vi "Configure.vi"(4 "Results Folder":path, 5 "Verdict Display":refnum<vi>, 6 "Stopped Notification":refnum<notifier>, 7 "Step Table Display":refnum<vi>, 8 "error in":errorcluster, 9 "Step Index Display":refnum<vi>, 10 "Status Display":refnum<vi>, 11 "Sequence Executor in":refnum<class "Sequence Executor.lvclass">) -> (0 "error out":errorcluster, 3 "Sequence Executor out":refnum<class "Sequence Executor.lvclass">)   [LabVIEW 2026, in "Sequence Executor.lvclass"]
doc: "Stores the UI display references, the Stopped Notification and the results folder in the actor's private data. Call it on the actor object BEFORE Launch Root Actor. Plant displays are stored by Configure Plant Displays.vi. Unwired (null) references are allowed: display writes ignore their errors."
uses:
  Sequence Executor.lvclass
  Sequence Executor.lvclass/Sequence Executor.ctl
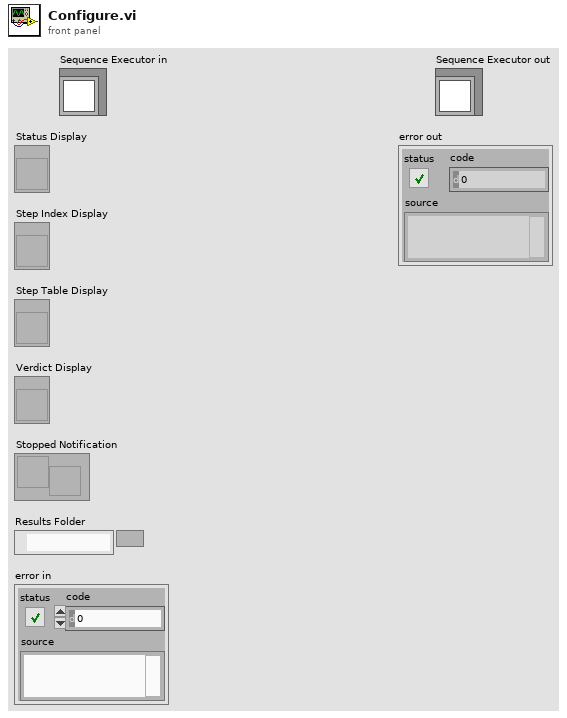
[diagram p1: front panel]
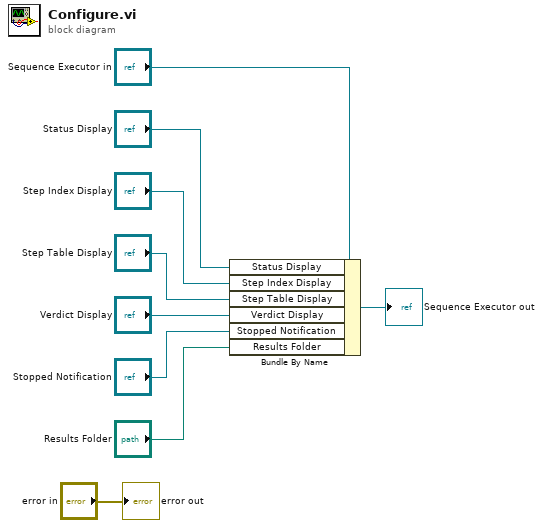
[diagram p0: block diagram]
diagram:
  n1 = Bundle By Name(cluster="Sequence Executor in", "Status Display"="Status Display", "Step Index Display"="Step Index Display", "Step Table Display"="Step Table Display", "Verdict Display"="Verdict Display", "Stopped Notification"="Stopped Notification", "Results Folder"="Results Folder") -> (→"Sequence Executor out":refnum<class "Sequence Executor.lvclass">)
  "error out" <- "error in"
